vi "PhotonCamera_SetDriverMode.vi"(9 "DriverMode":bool, 10 "BaseNTName":string="/photonvision", 11 "CameraName":string) -> (0 "error out":errorcluster)   [LabVIEW 2019, in "PhotonVisionLib.lvlib"]
doc: "Toggles driver mode.\n \nInputs:\n - cameraName -- The nickname of the camera (found in the PhotonVision UI).\n - BaseNTName - string - Base Nework Table name. (Optional. Default: /photonvision )\n - DriverMode -- Whether to set driver mode.\n\nOutputs:\n - Error Out -- Contains error information if a Network table ot other error occured."
uses:
  PhotonVisionLib.lvlib
  <vilib>/Rock Robotics/WPI/ThirdParty/JAS_Junk/TrajLib/VI/Util_GetTime_U32.vi
  <vilib>/Rock Robotics/WPI/ThirdParty/JAS_Junk/TrajLib/VI/Util_GetTime_U64.vi
  <vilib>/Rock Robotics/Network Tables/NT Read Boolean.vi
  <vilib>/Rock Robotics/Network Tables/NT Write Boolean.vi
  <vilib>/Rock Robotics/WPI/ThirdParty/JAS_Junk/TrajLib/Trajectory_Library.lvlib
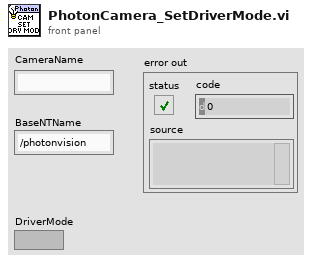
[diagram p1: front panel]
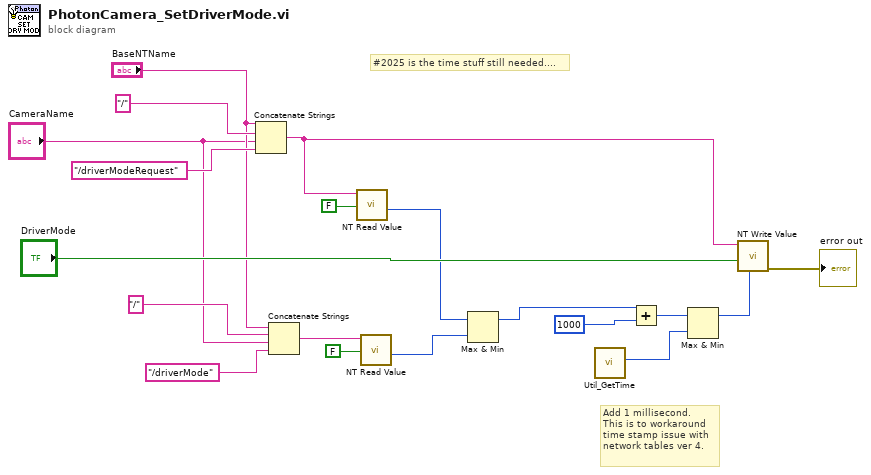
[diagram p0: block diagram]
diagram:
  # "#2025 is the time stuff still needed...."
  # "Add 1 millisecond.\nThis is to workaround\ntime stamp issue with\nnetwork tables ver 4."
  n1 = Concatenate Strings("BaseNTName", "/", "CameraName", "/driverModeRequest") -> (w15:string)
  n2 = Concatenate Strings("BaseNTName", "/", "CameraName", "/driverMode") -> (w7:string)
  n3 = call-poly <vilib>:"NT Read Value.vi"("default value"=FALSE ("Default Value"), "name"=w15) -> ("timestamp"=w2:u64)  [unwired: 7 in, 2 out]
  n4 = call-poly <vilib>:"NT Read Value.vi"("default value"=FALSE ("Default Value"), "name"=w7) -> ("timestamp"=w3:u64)  [unwired: 7 in, 2 out]
  n5 = Max & Min(x=w2, y=w3) -> (max(x,y)=w1:u64)  [unwired: 1 out]
  n6 = call <vilib>:"Util_GetTime.vi"() -> ("FPGA_Time_MicroSeconds"=w11:u64)  [unwired: 9 in, 2 out]
  n7 = Add(x=w1, y=u64 1000) -> (x+y=w13:u64)
  n8 = Max & Min(x=w13, y=w11) -> (max(x,y)=w12:u64)  [unwired: 1 out]
  n9 = call-poly <vilib>:"NT Write Value.vi"("timestamp"=w12, "value"="DriverMode", "name"=w15) -> ("error out"=→"error out":errorcluster)  [unwired: 8 in]
